vi "Diagnostics.vi"(8 "error in (no error)":errorcluster, 10 "pending bytes":string, 11 "data in":string) -> (0 "error out":errorcluster, 2 "decoded_frames":T1[](array[typedef]), 3 "remaining bytes":string)   [LabVIEW 2015, in "Lengmur_socket.lvlib"]
uses:
  Lengmur_socket.lvlib
  Types/Decoded Frame.ctl
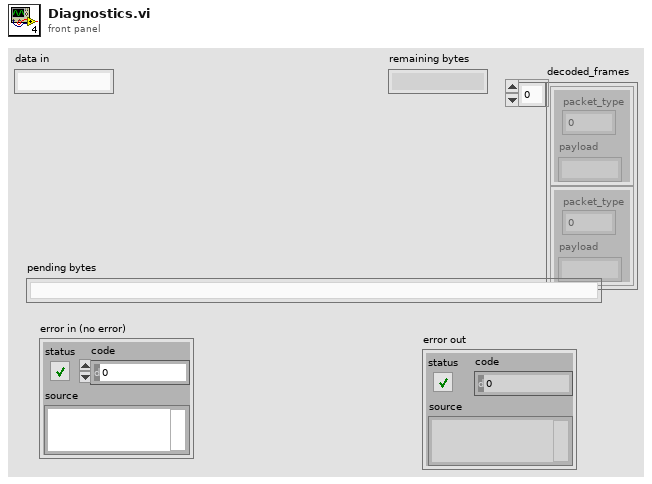
[diagram p1: front panel]
types:
  T1 = typedef "Lengmur_socket.lvlib/Decoded Frame.ctl" = cluster{"packet_type":u8, "payload":string}
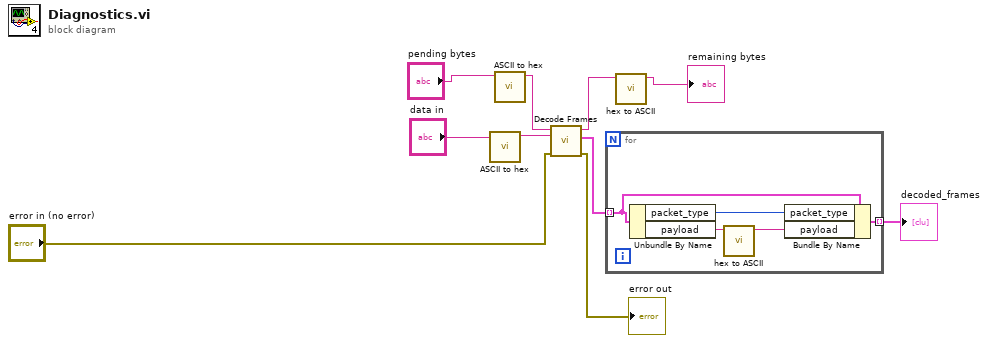
[diagram p0: block diagram]
diagram:
  n1 = call "ASCII to hex.vi"("ASCII string"="data in") -> ("hex string"=w7:string)  [unwired: 10 in]
  n2 = call "ASCII to hex.vi"("ASCII string"="pending bytes") -> ("hex string"=w9:string)  [unwired: 10 in]
  n3 = call "Decode Frames.vi"("error in"="error in (no error)", "data in"=w7, "pending bytes"=w9) -> ("error out"=→"error out":errorcluster, "decoded frames"=w4:T1[], "remaining bytes"=w6:string)  [unwired: 6 in]
  n4 = for {
    tunnel: w4 -> [w15] mode=indexing
    tunnel: [w11] -> w3 mode=indexing
    n5 = Unbundle By Name(w15) -> ("packet_type"=w14:u8, "payload"=w13:string)
    n6 = call "hex to ASCII.vi"("hex string"=w13) -> ("ASCII string"=w12:string)  [unwired: 10 in]
    n7 = Bundle By Name(cluster=w15, "packet_type"=w14, "payload"=w12) -> (w11:T1)
  }
  "decoded_frames" <- w3
  n8 = call "hex to ASCII.vi"("hex string"=w6) -> ("ASCII string"=→"remaining bytes":string)  [unwired: 10 in]
